vi "UMLEditor Main.vi"(1 "StartProject":string, 3 "StartTarget":string) -> ()   [LabVIEW 2020] (continued)
            n161 = call <resource>:"UndoEngine.vi"("Reference In"=w358, "Action"=enum16{"TakeSnapshot", "Undo", "Redo"}."TakeSnapshot", "Reset"=TRUE, "error in (no error)"=w357, "menu"=w356) -> ("Reference Out"=w355:refnum<class "Graph.lvclass">, "error out"=w354:errorcluster)  [unwired: 3 in, 10 out]
            n162 = Path To String(path=w368) -> (string=w367:string)
            n163 = call-dynamic "GetToolbarButtons.vi"("reference"=w355, "error in (no error)"=w354) -> ("AllToolbarButtons"=w351:T36[], "error out"=w353:errorcluster)  [unwired: 13 in, 3 out]
            n164 = case shown="False" w365 {
              tunnel: w367 -> [w373 _]
              tunnel: [w373 w374] -> w364
              tunnel: w363 -> [_ w374]
              frame False {
              }
              frame True {
              }
            }
            n165 = local write "GraphButtons"(T1."1" ("GraphButtons")) -> ()
            n166 = call <resource>:"UpdateToolbar.vi"("ToolbarButtons"=w351, "error in (no error)"=w353) -> ("error out"=w352:errorcluster)  [unwired: 17 in]
            n167 = property on="Diagram" class="Ring (strict)"("Tip Strip"=w364) -> ()  [unwired: 2 in, 2 out]
          }
          event "GraphButtons": Value Change {
            n168 = event-data() -> ()  [unwired: 7 out]
            n169 = call-dynamic "GetToolbarButtons.vi"("reference"=w378, "GraphButton"="GraphButtons", "error in (no error)"=w379) -> ("Type"=w376:T7, "error out"=w377:errorcluster)  [unwired: 12 in, 3 out]
            n170 = Bundle By Name(cluster=w381, "toolType"=w376) -> (w380:T5)
          }
          event "Help": Mouse Enter {
            n171 = event-data() -> ()  [unwired: 5 out]
            n172 = Unbundle By Name(w385) -> ("ToolHelp"=w384:bool)
            n173 = local read "Help"() -> (w383:bool)
            n174 = And(x=w384, y=w383) -> (x .and. y?=w382:bool)
            n175 = case shown="True" w382 {
              tunnel: w387 -> [w388 w391]
              tunnel: [w388 w390] -> w386
              frame False {
              }
              frame True {
                n176 = call <resource>:"ContextHelp_HelpTexts.vi"("HelpText (enum or string)"=ContextHelp_HelpTexts."Help" ("HelpText")) -> ("HelpOut"=w392:T38)  [unwired: 18 out]
                n177 = call <resource>:"ContextHelp_SendMessageToPopUp.vi"("PopUpMessage"=w392, "error in (no error)"=w391) -> ("error out"=w390:errorcluster)  [unwired: 1 in, 16 out]
              }
            }
          }
          event "Help": Value Change {
            n178 = event-data() -> ()  [unwired: 7 out]
            n179 = case shown="True" "Help" {
              tunnel: [ContextHelp_HelpTexts."None(Hide)" ("HelpText") ContextHelp_HelpTexts."Default" ("HelpText")] -> w395
              frame False {
              }
              frame True {
              }
            }
            n180 = call <resource>:"ContextHelp_HelpTexts.vi"("HelpText (enum or string)"=w395) -> ("HelpOut"=w398:T38)  [unwired: 18 out]
            n181 = call <resource>:"ContextHelp_SendMessageToPopUp.vi"("PopUpMessage"=w398, "error in (no error)"=w397) -> ("error out"=w396:errorcluster)  [unwired: 1 in, 16 out]
          }
          event "open": Value Change {
            n182 = event-data() -> ()  [unwired: 6 out]
            n183 = Bundle By Name(cluster=w402, "state"=UMLEditor_statesType."Open") -> (w403:T5)
          }
          event "Picture": Drag Enter {
            n184 = event-data() -> ("Coords"=w406:T39, "Available Data Names"=w405:string[])  [unwired: 8 out]
            n185 = stacked-sequence {
              tunnel: w406 -> [_]
              tunnel: w405 -> [_]
              frame #0 {
              }
            }
            n186 = event-data("Accepted?"=TRUE) -> ()  [unwired: 1 in, 1 out]
          }
          event "Picture": Mouse Down {
            # "Shift"
            n187 = event-data() -> ("Source"=w422:T40, "Button"=w416:u16, "Mods.Double Click"=w413:bool, "PlatMods.Ctrl"=w412:bool, "PlatMods.Shift"=w411:bool)  [unwired: 1 out]
            n188 = case shown="1, Default" w416 {
              selector: w416 -> [w453 _]
              tunnel: w422 -> [_ _]
              tunnel: w421 -> [w429 _]
              tunnel: [w462 w861] -> w420
              tunnel: w419 -> [w461 _]
              tunnel: w418 -> [w425 w860]
              tunnel: w410 -> [w452 w861]
              tunnel: [w454 w860] -> w417
              tunnel: w413 -> [w442 _]
              tunnel: w412 -> [w441 _]
              tunnel: w414 -> [_ _]
              tunnel: w411 -> [w433 _]
              frame 1, Default {
                n189 = local read "GraphButtons"() -> (w427:T1)
                n190 = call-dynamic "GetToolbarButtons.vi"("reference"=w429, "GraphButton"=w427, "error in (no error)"=w425) -> ("reference out"=w428:refnum<class "Graph.lvclass">, "Type"=w424:T7, "error out"=w426:errorcluster)  [unwired: 12 in, 2 out]
                n191 = property on="Picture" class="Pict"() -> ("Mouse"=w446:T41, "Draw Area Size"=w445:T42, "Origin"=w443:T43)  [unwired: 2 in, 2 out]
                n192 = Unbundle By Name(w452) -> ("graphics"=w436:refnum<class "Graphics.lvclass">, "SelectedNodes"=w448:refnum<class "AbstractNode.lvclass">[])
                n193 = Unbundle By Name(w452) -> ("HotSpotNode"=w430:refnum<class "AbstractNode.lvclass">, "HotSpotCursor"=w431:bool, "HotSpotFunction"=w432:T16, "zoom"=w455:dbl, "offset"=w457:T9)
                n194 = Unbundle By Name(w446) -> ("Mouse Position"=w458:cluster{"X":i32, "Y":i32})
                n195 = Array Size(array=w448) -> (size(s)=w450:i32)
                n196 = Greater?(x=w450, y=1) -> (0:w451:bool)
                n197 = Add(x=w457, y=w458) -> (x+y=w456:T9)
                n198 = call <resource>:"UMLEditor IsMouseOutsideDrawingArea.vi"("Mouse"=w446, "Draw Area Size"=w445, "Origin"=w443) -> ("OutsideDrawingArea"=w444:bool)  [unwired: 2 in, 14 out]
                n199 = Divide(x=w456, y=w455) -> (x/y=w440:T9)
                n200 = Bundle By Name(cluster=w452, "state"=UMLEditor_statesType."Repaint", "lastMousePoint"=w440) -> (w460:T5)
                n201 = call <resource>:"UMLEditor_FindObject.vi"("offset"=w440, "error in"=w426, "graphics"=w436, "graph"=w428) -> ("error out"=w439:errorcluster, "NodeFound"=w438:bool, "node"=w437:refnum<class "AbstractNode.lvclass">, "edge"=w435:refnum<class "AbstractEdge.lvclass">, "EdgeFound"=w434:bool)  [unwired: 2 in, 1 out]
                n202 = Tick Count (ms)() -> (millisecond timer value=w447:u32)
                n203 = case shown="False" w444 {
                  tunnel: w439 -> [w492 w859]
                  tunnel: w438 -> [w468 _]
                  tunnel: w434 -> [w477 _]
                  tunnel: w435 -> [w491 _]
                  tunnel: w437 -> [w490 _]
                  tunnel: [w489 w857] -> w462
                  tunnel: w461 -> [w487 _]
                  tunnel: w424 -> [w486 _]
                  tunnel: w428 -> [w485 _]
                  tunnel: w460 -> [w484 w858]
                  tunnel: w440 -> [w483 _]
                  tunnel: [w482 w859] -> w454
                  tunnel: w453 -> [w481 _]
                  tunnel: w451 -> [w480 _]
                  tunnel: w448 -> [w479 _]
                  tunnel: w447 -> [_ _]
                  tunnel: w445 -> [_ _]
                  tunnel: w442 -> [w469 _]
                  tunnel: w441 -> [w474 _]
                  tunnel: w436 -> [w472 _]
                  tunnel: w433 -> [w467 _]
                  tunnel: w432 -> [_ _]
                  tunnel: w431 -> [w465 _]
                  tunnel: w430 -> [w464 _]
                  tunnel: w427 -> [w463 _]
                  frame False {
                    n204 = Or(x=w468, y=w477) -> (x .or. y?=w476:bool)
                    n205 = And(x=w468, y=w467) -> (x .and. y?=w466:bool)
                    n206 = Compound Arithmetic op=AND(w469, w476) -> (w478:bool)
                    n207 = case shown="True" w478 {
                      tunnel: w492 -> [w509 w808]
                      tunnel: [w508 w807] -> w482
                      tunnel: w468 -> [w511 w806]
                      tunnel: w477 -> [w502 w801]
                      tunnel: w486 -> [w501 _]
                      tunnel: w484 -> [w514 w805]
                      tunnel: [w513 w804] -> w488
                      tunnel: w491 -> [w512 w803]
                      tunnel: w490 -> [w510 w802]
                      tunnel: w483 -> [w507 w799]
                      tunnel: w487 -> [w506 _]
                      tunnel: w485 -> [w505 _]
                      tunnel: w481 -> [_ _]
                      tunnel: w480 -> [w504 _]
                      tunnel: w479 -> [w503 _]
                      tunnel: UMLEditor_tooltype."None" ("t") -> [w500 _]
                      tunnel: w474 -> [w497 w800]
                      tunnel: [TRUE ("butDwn") w798] -> w473
                      tunnel: w472 -> [w498 _]
                      tunnel: w466 -> [w496 _]
                      tunnel: [w496 w798] -> w471
                      tunnel: [w497 w798] -> w470
                      tunnel: w469 -> [_ _]
                      tunnel: w465 -> [w495 _]
                      tunnel: w464 -> [w494 _]
                      tunnel: w463 -> [w493 _]
                      frame False {
                        # "Single Click"
                        n208 = case shown="True" w496 {
                          tunnel: w514 -> [w534 w786]
                          tunnel: [w533 w785] -> w513
                          tunnel: w512 -> [w532 _]
                          tunnel: w511 -> [w531 _]
                          tunnel: w510 -> [w530 w782]
                          tunnel: w509 -> [w529 w781]
                          tunnel: [w528 w781] -> w508
                          tunnel: w507 -> [w527 w784]
                          tunnel: w506 -> [w526 _]
                          tunnel: w505 -> [w525 _]
                          tunnel: w504 -> [w524 _]
                          tunnel: w503 -> [w523 w783]
                          tunnel: w502 -> [w522 _]
                          tunnel: w501 -> [w521 _]
                          tunnel: w500 -> [w519 _]
                          tunnel: w498 -> [w518 _]
                          tunnel: [_ w779] -> _
                          tunnel: w495 -> [w517 _]
                          tunnel: w494 -> [w516 _]
                          tunnel: w493 -> [w515 _]
                          frame False {
                            n209 = Select(t=w519, s=w522, f=w521) -> (s? t:f=w520:T7)
                            n210 = case shown="True" w517 {
                              tunnel: w534 -> [w551 w771]
                              tunnel: [w550 w770] -> w533
                              tunnel: w532 -> [w549 _]
                              tunnel: w531 -> [w548 _]
                              tunnel: w530 -> [w547 _]
                              tunnel: w529 -> [w546 w773]
                              tunnel: [w545 w772] -> w528
                              tunnel: w527 -> [w544 w769]
                              tunnel: w526 -> [w543 _]
                              tunnel: w525 -> [w542 _]
                              tunnel: w524 -> [w541 _]
                              tunnel: w523 -> [w540 _]
                              tunnel: w522 -> [w539 _]
                              tunnel: w520 -> [w538 _]
                              tunnel: w518 -> [w537 _]
                              tunnel: w517 -> [w536 _]
                              tunnel: w516 -> [_ w768]
                              tunnel: w515 -> [w535 _]
                              frame False {
                                n211 = case shown="\"None\", Default" w538 {
                                tunnel: w539 -> [w565 _ _]
                                tunnel: w551 -> [w564 w700 w747]
                                tunnel: [w563 w699 w746] -> w550
                                tunnel: w549 -> [w562 _ _]
                                tunnel: w548 -> [w561 w696 w744]
                                tunnel: w547 -> [w560 w695 w743]
                                tunnel: w546 -> [w559 w693 w742]
                                tunnel: [w558 w697 w741] -> w545
                                tunnel: w544 -> [w557 w694 w745]
                                tunnel: w543 -> [_ _ w740]
                                tunnel: w542 -> [w556 w692 w739]
                                tunnel: w541 -> [w555 _ _]
                                tunnel: w540 -> [w554 _ _]
                                tunnel: w537 -> [w553 _ _]
                                tunnel: w536 -> [w552 _ _]
                                tunnel: w535 -> [_ w691 w738]
                                frame "None", Default {
                                # "Select"
                                n212 = case shown="False" w565 {
                                tunnel: w564 -> [w574 w667]
                                tunnel: [w573 w666] -> w563
                                tunnel: w562 -> [_ w630]
                                tunnel: w561 -> [w575 _]
                                tunnel: w560 -> [w572 _]
                                tunnel: w559 -> [w571 w646]
                                tunnel: [w570 w646] -> w558
                                tunnel: w557 -> [w569 w641]
                                tunnel: w556 -> [_ _]
                                tunnel: w555 -> [w568 _]
                                tunnel: w554 -> [w567 _]
                                tunnel: w553 -> [_ w627]
                                tunnel: w552 -> [w566 _]
                                frame False {
                                n213 = case shown="True" w575 {
                                tunnel: w574 -> [w579 w625]
                                tunnel: [w584 w624] -> w573
                                tunnel: w572 -> [w585 _]
                                tunnel: w571 -> [w586 w621]
                                tunnel: [w583 w621] -> w570
                                tunnel: w569 -> [w582 w618]
                                tunnel: w568 -> [w581 _]
                                tunnel: w567 -> [w580 _]
                                tunnel: w566 -> [w576 _]
                                frame True {
                                # "Node Selected"
                                n214 = case shown="False" w576 {
                                frame False {
                                n215 = call <resource>:"UMLEditor_SetMouseCursor.vi"("CursorType"=UMLEditor_Cursortype."Move") -> ()  [unwired: 9 in, 2 out]
                                }
                                frame True {
                                }
                                }
                                n216 = Bundle By Name(cluster=w579, "state"=UMLEditor_statesType."Idle") -> (w577:T5)
                                n217 = case shown="False" w581 {
                                tunnel: w586 -> [w597 w601]
                                tunnel: w585 -> [w596 w600]
                                tunnel: w577 -> [w593 w599]
                                tunnel: [w592 w605] -> w584
                                tunnel: [w590 w601] -> w583
                                tunnel: w582 -> [w588 w604]
                                tunnel: w580 -> [_ w603]
                                frame False {
                                n218 = call-dynamic "getBounds.vi"("reference"=w596, "error in (no error)"=w597) -> ("reference out"=w595:refnum<class "AbstractNode.lvclass">, "bounds"=w594:T10, "error out"=w590:errorcluster)  [unwired: 15 in]
                                n219 = Build Array(w595) -> (w589:refnum<class "AbstractNode.lvclass">[])
                                n220 = Bundle By Name(cluster=w593, "selected"=UMLEditor_tooltype."Node" ("selcted"), "SelectedNodes"=w589, "dragStartBounds"=w594, "dragStartPoint"=w588, "newSelected"=TRUE, "lastMousePoint"=w588) -> (w592:T5)
                                }
                                frame True {
                                # "If many nodes allready selected move these"
                                n221 = Search 1D Array(1D array=w603, element=w600) -> (index of element=w602:i32)  [unwired: 1 out]
                                n222 = case shown="-1" w602 {
                                tunnel: w599 -> [w610 w617]
                                tunnel: [w609 w616] -> w605
                                tunnel: w604 -> [w608 w615]
                                tunnel: w600 -> [_ w612]
                                frame Default {
                                n223 = Bundle By Name(cluster=w610, "selected"=UMLEditor_tooltype."Node" ("selcted"), "dragStartPoint"=w608, "newSelected"=TRUE, "lastMousePoint"=w608) -> (w609:T5)
                                }
                                frame -1 {
                                n224 = Build Array(w612) -> (w611:refnum<class "AbstractNode.lvclass">[])
                                n225 = Bundle By Name(cluster=w617, "selected"=UMLEditor_tooltype."Node" ("selcted"), "dragStartPoint"=w615, "newSelected"=TRUE, "lastMousePoint"=w615, "SelectedNodes"=w611) -> (w616:T5)
                                }
                                }
                                }
                                }
                                }
                                frame False {
                                # "None Selected\nArea Select???"
                                n226 = Bundle By Name(cluster=w625, "selected"=UMLEditor_tooltype."None" ("selcted"), "SelectedNodes"=refnum<class "AbstractNode.lvclass">[] [], "dragStartBounds"=T10 {"x"=0.0, "y"=0.0, "width"=0.0, "height"=0.0}, "dragStartPoint"=w618, "rubberBandStart"=w618, "newSelected"=TRUE, "state"=UMLEditor_statesType."Idle", "lastMousePoint"=w618) -> (w624:T5)
                                }
                                }
                                }
                                frame True {
                                w663 = 25.0 ("y")
                                n227 = To More Specific Class(target class=refnum<class "GeneralPathEdge.lvclass"> refnum ("reference"), reference=w630) -> (specific class reference=w628:refnum<class "GeneralPathEdge.lvclass">)  [unwired: 1 in, 1 out]
                                n228 = call-dynamic "getPoints.vi"("reference"=w628, "error in (no error)"=w646) -> ("reference out"=w644:refnum<class "GeneralPathEdge.lvclass">, "points"=w642:T9[], "error out"=w645:errorcluster)  [unwired: 15 in]
                                n229 = Array Size(array=w642) -> (size(s)=w643:i32)
                                n230 = case shown="4" w643 {
                                tunnel: w642 -> [_ w676]
                                tunnel: w641 -> [_ w671]
                                tunnel: [_ w668] -> w636
                                frame Default {
                                }
                                frame 4 {
                                # "Egde selected"
                                n231 = Index Array(array=w676, index #1=1 ("index")) -> (element #1=w674:T9, element #2=w673:T9)  [unwired: 1 in]
                                n232 = Build Array(w674, w673) -> (w672:T9[])
                                n233 = call <resource>:"Point getDistanceToLine.vi"("point1"=w671, "line"=w672) -> ("minDistance"=w670:dbl)  [unwired: 1 in, 16 out]
                                n234 = Less?(x=w670, y=25.0) -> (x < y?=w668:bool)
                                }
                                }
                                n235 = Index Array(array=w642) -> (element=w662:T9)  [unwired: 1 in]
                                n236 = Delete From Array(array=w642) -> (deleted portion=w661:T9)  [unwired: 2 in, 1 out]
                                n237 = call-dynamic "GetTextPositions.vi"("reference"=w644, "GraphicsRef"=w627, "error in (no error)"=w645) -> ("reference out"=w654:refnum<class "GeneralPathEdge.lvclass">, "connectionPoints"=w653:T9[], "error out"=w655:errorcluster)  [unwired: 14 in]
                                n238 = Index Array(array=w653) -> (element=w652:T9)  [unwired: 1 in]
                                n239 = call <resource>:"Point getDistance.vi"("point1"=w662, "point2"=w641) -> ("distance"=w665:dbl)  [unwired: 1 in, 16 out]
                                n240 = call <resource>:"Point getDistance.vi"("point1"=w661, "point2"=w641) -> ("distance"=w664:dbl)  [unwired: 1 in, 16 out]
                                n241 = call-dynamic "getEnd.vi"("reference"=w654, "error in (no error)"=w655) -> ("reference out"=w659:refnum<class "GeneralPathEdge.lvclass">, "endNode"=w633:refnum<class "AbstractNode.lvclass">, "error out"=w660:errorcluster)  [unwired: 14 in, 1 out]
                                n242 = call <resource>:"Point getDistance.vi"("point1"=w652, "point2"=w641) -> ("distance"=w651:dbl)  [unwired: 1 in, 16 out]
                                n243 = Less?(x=w664, y=w663) -> (x < y?=w639:bool)
                                n244 = Less?(x=w665, y=w663) -> (x < y?=w638:bool)
                                n245 = Less?(x=w651, y=40.0) -> (x < y?=w640:bool)
                                n246 = call-dynamic "getStart.vi"("reference"=w659, "error in (no error)"=w660) -> ("startNode"=w632:refnum<class "AbstractNode.lvclass">, "error out"=w658:errorcluster)  [unwired: 14 in, 2 out]
                                n247 = Select(t=w633, s=w639, f=w632) -> (s? t:f=w649:refnum<class "AbstractNode.lvclass">)
                                n248 = Unbundle By Name(w658) -> ("status"=w657:bool)
                                n249 = Build Array(w633, w632) -> (w631:refnum<class "AbstractNode.lvclass">[])
                                n250 = Compound Arithmetic op=OR(w636, w638, w639, w640) -> (w637:bool)
                                n251 = Build Array(w649) -> (w635:refnum<class "AbstractNode.lvclass">[])
                                n252 = Compound Arithmetic op=AND(w637, invert w657) -> (w656:bool)
                                n253 = Select(t=w631, s=w636, f=w635) -> (s? t:f=w634:refnum<class "AbstractNode.lvclass">[])
                                n254 = Select(t=refnum<class "AbstractNode.lvclass">[] [], s=w640, f=w634) -> (s? t:f=w647:refnum<class "AbstractNode.lvclass">[])
                                n255 = case shown="True" w656 {
                                tunnel: w667 -> [w683 w688]
                                tunnel: [w682 w687] -> w666
                                tunnel: w630 -> [w679 w684]
                                tunnel: w641 -> [w678 _]
                                tunnel: w647 -> [w677 _]
                                frame True {
                                n256 = Bundle By Name(cluster=w683, "selected"=UMLEditor_tooltype."Edge" ("selcted"), "selectedEdge"=w679, "dragStartPoint"=w678, "newSelected"=TRUE, "SelectedNodes"=w677) -> (w682:T5)
                                }
                                frame False {
                                n257 = Bundle By Name(cluster=w688, "selected"=UMLEditor_tooltype."Edge" ("selcted"), "selectedEdge"=w684, "newSelected"=TRUE) -> (w687:T5)
                                }
                                }
                                }
                                }
                                }
                                frame "Node" {
                                # "Node Tool"
                                n258 = call-dynamic "CreateToolbarObject.vi"("reference in"=w692, "GraphButton"=w691, "error in (no error)"=w693) -> ("Node"=w689:refnum<class "AbstractNode.lvclass">, "error out"=w690:errorcluster)  [unwired: 11 in, 4 out]
                                n259 = call-dynamic "add.vi"("reference"=w692, "node"=w689, "point"=w694, "error in (no error)"=w690) -> ("added"=w701:bool, "error out"=w698:errorcluster)  [unwired: 13 in, 1 out]
                                n260 = case shown="False" w701 {
                                tunnel: w700 -> [w709 w729]
                                tunnel: [w708 w727] -> w699
                                tunnel: w698 -> [w704 w737]
                                tunnel: w689 -> [w702 w736]
                                tunnel: w694 -> [w706 w725]
                                tunnel: [w705 w730] -> w697
                                tunnel: w696 -> [w710 _]
                                tunnel: w695 -> [w707 _]
                                frame False {
                                n261 = call-dynamic "Destroy.vi"("reference"=w702, "error in (no error)"=w704) -> ("error out"=w703:errorcluster)  [unwired: 16 in, 1 out]
                                n262 = case shown="True" w710 {
                                tunnel: w709 -> [w712 w721]
                                tunnel: [w712 w720] -> w708
                                tunnel: w703 -> [w711 w723]
                                tunnel: w707 -> [_ w715]
                                tunnel: w706 -> [_ w717]
                                tunnel: [w711 w719] -> w705
                                frame False {
                                }
                                frame True {
                                # "Node Found"
                                n263 = call-dynamic "getBounds.vi"("reference"=w715, "error in (no error)"=w723) -> ("bounds"=w722:T10, "error out"=w719:errorcluster)  [unwired: 15 in, 1 out]
                                n264 = Build Array(w715) -> (w718:refnum<class "AbstractNode.lvclass">[])
                                n265 = local write "GraphButtons"(T1."1" ("GraphButtons")) -> ()
                                n266 = Bundle By Name(cluster=w721, "selected"=UMLEditor_tooltype."Node" ("selcted"), "SelectedNodes"=w718, "dragStartBounds"=w722, "dragStartPoint"=w717, "lastMousePoint"=w717, "newSelected"=TRUE, "toolType"=UMLEditor_tooltype."None") -> (w720:T5)
                                }
                                }
                                }
                                frame True {
                                # "Added"
                                n267 = call-dynamic "getBounds.vi"("reference"=w736, "error in (no error)"=w737) -> ("reference out"=w734:refnum<class "AbstractNode.lvclass">, "bounds"=w735:T10, "error out"=w731:errorcluster)  [unwired: 15 in]
                                n268 = Build Array(w734) -> (w726:refnum<class "AbstractNode.lvclass">[])
                                n269 = Bundle By Name(cluster=w729, "selected"=UMLEditor_tooltype."Node" ("selcted"), "SelectedNodes"=w726, "dragStartBounds"=w735, "dragStartPoint"=w725, "lastMousePoint"=w725) -> (w728:T5)
                                n270 = call <resource>:"UMLEditor setDiagramInfo.vi"("error in (no error)"=w731, "localVariablesIn"=w728, "action"=enum16{"Name/Dir", "Unsaved", "Saved"}."Unsaved") -> ("localVariablesOut"=w727:T5, "error out"=w730:errorcluster)  [unwired: 2 in, 13 out]
                                }
                                }
                                }
                                frame "Edge" {
                                # "Edge Tool"
                                n271 = case shown="True" w744 {
                                tunnel: w747 -> [w750 w761]
                                tunnel: [w749 w760] -> w746
                                tunnel: w745 -> [_ w759]
                                tunnel: w743 -> [_ w758]
                                tunnel: w742 -> [w752 w757]
                                tunnel: [w752 w755] -> w741
                                tunnel: w740 -> [_ _]
                                tunnel: w739 -> [_ w754]
                                tunnel: w738 -> [_ w753]
                                frame False {
                                n272 = local write "GraphButtons"(T1."1" ("GraphButtons")) -> ()
                                n273 = Bundle By Name(cluster=w750, "toolType"=UMLEditor_tooltype."None") -> (w749:T5)
                                }
                                frame True {
                                n274 = call-dynamic "AllowEdgeStartCheck.vi"("reference in"=w754, "EdgeStartNode"=w758, "GraphButton"=w753, "error in (no error)"=w757) -> ("Allowed"=w756:bool, "error out"=w755:errorcluster)  [unwired: 13 in, 1 out]
                                n275 = case shown="True" w756 {
                                tunnel: w761 -> [w762 w767]
                                tunnel: [w762 w766] -> w760
                                tunnel: w759 -> [_ w765]
                                frame False {
                                }
                                frame True {
                                n276 = Bundle By Name(cluster=w767, "rubberBandStart"=w765, "selected"=UMLEditor_tooltype."Edge" ("selcted"), "state"=UMLEditor_statesType."Idle") -> (w766:T5)
                                }
                                }
                                }
                                }
                                }
                                }
                              }
                              frame True {
                                n277 = call-dynamic "getBounds.vi"("reference"=w768, "error in (no error)"=w773) -> ("reference out"=w777:refnum<class "AbstractNode.lvclass">, "bounds"=w776:T10, "error out"=w772:errorcluster)  [unwired: 15 in]
                                n278 = Build Array(w777) -> (w774:refnum<class "AbstractNode.lvclass">[])
                                n279 = Bundle By Name(cluster=w771, "selected"=UMLEditor_tooltype."Node" ("selcted"), "SelectedNodes"=w774, "dragStartBounds"=w776, "dragStartPoint"=w769, "newSelected"=TRUE, "lastMousePoint"=w769) -> (w770:T5)
                              }
                            }
                          }
                          frame True {
                            # "Shift Click"
                            n280 = Search 1D Array(1D array=w783, element=w782) -> (index of element=w791:i32)  [unwired: 1 in]
                            n281 = case shown="0, Default" w791 {
                              selector: w791 -> [w792 _]
                              tunnel: w783 -> [w794 w797]
                              tunnel: w782 -> [_ w796]
                              tunnel: [w793 w795] -> w780
                              frame 0, Default {
                                n282 = Delete From Array(array=w794, index=w792) -> (array with subset deleted=w793:refnum<class "AbstractNode.lvclass">[])  [unwired: 1 in, 1 out]
                              }
                              frame -1 {
                                n283 = Build Array (concatenate)(w797, w796) -> (w795:refnum<class "AbstractNode.lvclass">[])
                              }
                            }
                            n284 = Array Size(array=w780) -> (size(s)=w779:i32)
                            n285 = Bundle By Name(cluster=w786, "selected"=UMLEditor_tooltype."Node" ("selcted"), "SelectedNodes"=w780, "dragStartBounds"=T10 {"x"=nan, "y"=nan, "width"=nan, "height"=nan}, "dragStartPoint"=T9 {"x"=nan, "y"=nan}, "newSelected"=TRUE, "lastMousePoint"=w784) -> (w785:T5)
                          }
                        }
                      }
                      frame True {
                        w798 = FALSE ("butDwn")
                        # "DblClick"
                        n286 = case shown="True" w801 {
                          tunnel: w808 -> [w817 w851]
                          tunnel: [w816 w851] -> w807
                          tunnel: w806 -> [w815 _]
                          tunnel: w805 -> [w814 w853]
                          tunnel: [w813 w852] -> w804
                          tunnel: w803 -> [w812 w850]
                          tunnel: w802 -> [w811 _]
                          tunnel: w800 -> [w810 _]
                          tunnel: w799 -> [w809 _]
                          frame False {
                            n287 = case shown="False" w815 {
                              tunnel: w817 -> [w818 w823]
                              tunnel: [w818 w822] -> w816
                              tunnel: w814 -> [w819 w826]
                              tunnel: [w819 w825] -> w813
                              tunnel: w812 -> [_ _]
                              tunnel: w811 -> [_ w820]
                              tunnel: w810 -> [_ w824]
                              tunnel: w809 -> [_ w821]
                              frame False {
                              }
                              frame True {
                                # "Node Found"
                                n288 = case shown="True" w824 {
                                tunnel: w826 -> [w831 w838]
                                tunnel: [w830 w837] -> w825
                                tunnel: w820 -> [w828 _]
                                tunnel: w823 -> [w827 w842]
                                tunnel: [w827 w841] -> w822
                                tunnel: w821 -> [_ w840]
                                tunnel: w820 -> [_ w839]
                                frame False {
                                n289 = Build Array(w828) -> (w829:refnum<class "AbstractNode.lvclass">[])
                                n290 = Bundle By Name(cluster=w831, "selected"=UMLEditor_tooltype."Node" ("selcted"), "SelectedNodes"=w829, "state"=UMLEditor_statesType."EditSelected") -> (w830:T5)
                                }
                                frame True {
                                n291 = call-dynamic "GetContextHelpInfo.vi"("reference"=w839, "MousePos"=w840, "error in (no error)"=w842) -> ("ContextHelpInfo"=w836:variant, "error out"=w841:errorcluster)  [unwired: 13 in, 2 out]
                                n292 = Variant To Data(type=path "", Variant=w836) -> (error out=w834:errorcluster)  [unwired: 1 in, 1 out]
                                n293 = case shown="No Error" w834 {
                                tunnel: w838 -> [w847 w849]
                                tunnel: [w846 w849] -> w837
                                tunnel: w836 -> [w843 _]
                                frame No Error {
                                # "Ctrl-Key down\nSo lets open the method"
                                n294 = Bundle By Name(cluster=T12 {"Command"=enum."OpenFile", "CommandData"=variant} ("FlattenCommandSettings"), "CommandData"=w843) -> (w844:T12)
                                n295 = Bundle By Name(cluster=w847, "state"=UMLEditor_statesType."ExecuteCommand", "FlattenCommandSettings"=w844) -> (w846:T5)
                                }
                                frame Error {
                                }
                                }
                                }
                                }
                              }
                            }
                          }
                          frame True {
                            # "Edge Found"
                            n296 = Bundle By Name(cluster=w853, "selected"=UMLEditor_tooltype."Edge" ("selcted"), "selectedEdge"=w850, "state"=UMLEditor_statesType."EditSelected") -> (w852:T5)
                          }
                        }
                      }
                    }
                    n297 = Bundle By Name(cluster=w488, "butDwn"=w473, "ShiftDown"=w471, "CtrlDown"=w470) -> (w489:T5)
                  }
                  frame True {
                    # "SCROLLING"
                    n298 = Bundle By Name(cluster=w858, "state"=UMLEditor_statesType."Idle") -> (w857:T5)
                  }
                }
              }
              frame 0, 2 {
              }
            }
            n299 = property on="ClassAggregationDialog" class="Clust (strict)"() -> ("Visible"=w415:bool)  [unwired: 2 in, 2 out]
            n300 = case shown="True" w415 {
              frame False {
              }
              frame True {
                n301 = property on="ClassAggregationDialog" class="Clust (strict)"("Visible"=FALSE) -> ()  [unwired: 2 in, 2 out]
              }
            }
          }
          event "Picture": Mouse Enter {
            n302 = event-data() -> ()  [unwired: 5 out]
            n303 = call <resource>:"UMLEditor_SetMouseCursor.vi"("CursorType"=UMLEditor_Cursortype."Arrow") -> ("error out"=w863:errorcluster)  [unwired: 9 in, 1 out]
            n304 = property on="Picture" class="Pict"(error in=w863, "Cursor"=0) -> ()  [unwired: 1 in, 2 out]
          }
          event "Picture": Mouse Leave {
            n305 = event-data() -> ()  [unwired: 5 out]
            n306 = Unbundle By Name(w872) -> ("butDwn"=w871:bool)
            n307 = call <resource>:"UMLEditor_SetMouseCursor.vi"("CursorType"=UMLEditor_Cursortype."Arrow") -> ()  [unwired: 9 in, 2 out]
            n308 = Select(t=UMLEditor_statesType."Repaint" ("state"), s=w871, f=UMLEditor_statesType."Idle" ("state")) -> (s? t:f=w870:T6)
            n309 = Bundle By Name(cluster=w872, "state"=w870) -> (w873:T5)
          }
          event "Picture": Mouse Up {
            w905 = T9 {"x"=nan, "y"=nan} ("rubberBandStart")
            w880 = FALSE ("b_dwn")
            n310 = event-data() -> ("Mods.Double Click"=w893:bool, "Coords"=w888:T39)  [unwired: 1 out]
            n311 = Unbundle By Name(w875) -> ("lastMousePoint"=w879:T9, "rubberBandStart"=w901:T9, "selected"=w896:T7, "offset"=w884:T9, "zoom"=w882:dbl)
            n312 = Unbundle By Name(w875) -> ("SelectedNodes"=w894:refnum<class "AbstractNode.lvclass">[])
            n313 = Unbundle By Name(w875) -> ("HotSpotCursor"=w887:bool, "HotSpotFunction"=w886:T16)
            n314 = Unbundle By Name(w875) -> ("CONNECT_THRESHOLD"=w900:i32)
            n315 = property on="Picture" class="Pict"() -> ("Mouse"=w878:T41, "Draw Area Size"=w890:T42, "Origin"=w889:T43)  [unwired: 2 in, 2 out]
            n316 = Unbundle By Name(w878) -> ("Mouse Position"=w885:cluster{"X":i32, "Y":i32})
            n317 = call <resource>:"UMLEditor_SetMouseCursor.vi"("CursorType"=UMLEditor_Cursortype."Arrow") -> ()  [unwired: 9 in, 2 out]
            n318 = Tick Count (ms)() -> (millisecond timer value=w892:u32)
            n319 = Add(x=w885, y=w884) -> (x+y=w883:T9)
            n320 = call <resource>:"UMLEditor IsMouseOutsideDrawingArea.vi"("Mouse"=w878, "Draw Area Size"=w890, "Origin"=w889) -> ("OutsideDrawingArea"=w891:bool)  [unwired: 2 in, 14 out]
            n321 = call <resource>:"Point getValues.vi"("point2D"=w901) -> ("valid"=w903:bool)  [unwired: 18 out]
            n322 = Divide(x=w883, y=w882) -> (x/y=w881:T9)
            n323 = case shown="False" w891 {
              tunnel: w903 -> [w923 _]
              tunnel: w902 -> [w922 w1197]
              tunnel: w901 -> [w921 _]
              tunnel: w900 -> [w920 _]
              tunnel: [w909 w1196] -> w899
              tunnel: w898 -> [w919 _]
              tunnel: [w918 w1197] -> w897
              tunnel: w896 -> [w917 _]
              tunnel: w875 -> [w916 w1196]
              tunnel: UMLEditor_tooltype."None" ("y") -> [w915 _]
              tunnel: w894 -> [w914 _]
              tunnel: w893 -> [w913 _]
              tunnel: w892 -> [w912 _]
              tunnel: w888 -> [w911 _]
              tunnel: w887 -> [w910 _]
              tunnel: w886 -> [w908 _]
              tunnel: w881 -> [w907 _]
              tunnel: w879 -> [w906 _]
              frame False {
                n324 = case shown="False" w910 {
                  tunnel: w923 -> [w939 _]
                  tunnel: w922 -> [w938 w1151]
                  tunnel: w921 -> [w937 _]
                  tunnel: w920 -> [w936 _]
                  tunnel: w919 -> [w934 w1147]
                  tunnel: [w933 w1154] -> w918
                  tunnel: w917 -> [w932 _]
                  tunnel: w916 -> [w931 w1153]
                  tunnel: w915 -> [w930 _]
                  tunnel: w914 -> [w929 w1150]
                  tunnel: w913 -> [w928 _]
                  tunnel: w912 -> [w927 _]
                  tunnel: w911 -> [w926 _]
                  tunnel: [w935 w1152] -> w909
                  tunnel: w908 -> [_ w1149]
                  tunnel: w907 -> [w925 w1148]
                  tunnel: w906 -> [w924 _]
                  frame False {
                    n325 = case shown="False" w939 {
                      tunnel: w938 -> [w952 w1047]
                      tunnel: w931 -> [w953 w1046]
                      tunnel: w937 -> [_ w1042]
                      tunnel: w936 -> [_ w1045]
                      tunnel: w931 -> [w949 w1040]
                      tunnel: [w948 w1044] -> w935
                      tunnel: w934 -> [w950 w1043]
                      tunnel: [w951 w1041] -> w933
                      tunnel: w932 -> [w947 w1039]
                      tunnel: w930 -> [w944 _]
                      tunnel: w929 -> [w943 _]
                      tunnel: w928 -> [w942 _]
                      tunnel: w927 -> [_ _]
                      tunnel: w926 -> [_ w1038]
                      tunnel: w925 -> [w941 w1037]
                      tunnel: w924 -> [w940 _]
                      frame False {
                        # "Try to lock Assoc to grid is offset is used"
                        n326 = Not Equal?(x=w947, y=w944) -> (x != y?=w946:bool)
                        n327 = And(x=w946, y=w942) -> (x .and. y?=w945:bool)
                        n328 = case shown="False" w945 {
                          tunnel: w947 -> [w964 w1026]
                          tunnel: w953 -> [w963 _]
                          tunnel: w952 -> [w962 w1028]
                          tunnel: [w961 w1028] -> w951
                          tunnel: w950 -> [w960 _]
                          tunnel: w949 -> [w959 w1030]
                          tunnel: [w958 w1029] -> w948
                          tunnel: w943 -> [w957 w1027]
                          tunnel: w941 -> [w956 _]
                          tunnel: w941 -> [w955 _]
                          tunnel: w940 -> [w954 _]
                          frame False {
                            n329 = case shown="\"Edge\"" w964 {
                              tunnel: w963 -> [_ w977 _]
                              tunnel: w962 -> [w966 w976 w984]
                              tunnel: [w966 w974 w985] -> w961
                              tunnel: w960 -> [_ w973 w982]
                              tunnel: w959 -> [w965 w969 w987]
                              tunnel: [w965 w968 w986] -> w958
                              tunnel: w957 -> [_ _ w981]
                              tunnel: w956 -> [_ _ w983]
                              tunnel: w955 -> [_ _ w980]
                              tunnel: w954 -> [_ _ w979]
                              frame Default {
                              }
                              frame "Edge" {
                                n330 = Unbundle By Name(w977) -> ("selectedEdge"=w975:refnum<class "AbstractEdge.lvclass">, "graphics"=w972:refnum<class "Graphics.lvclass">, "grid"=w971:refnum<class "Grid.lvclass">)
                                n331 = call-dynamic "Layout.vi"("reference"=w975, "graph"=w973, "graphics"=w972, "grid"=w971, "error in (no error)"=w976) -> ("error out"=w974:errorcluster)  [unwired: 13 in, 1 out]
                                n332 = Bundle By Name(cluster=w969, "SelectedNodes"=refnum<class "AbstractNode.lvclass">[] [], "state"=UMLEditor_statesType."Repaint") -> (w968:T5)
                              }
                              frame "Node" {
                                n333 = case shown="True" TRUE {
                                tunnel: [w989 w1000] -> w985
                                tunnel: w984 -> [w989 w999]
                                tunnel: w983 -> [_ w998]
                                tunnel: w982 -> [_ w996]
                                tunnel: w981 -> [_ w990]
                                frame False {
                                }
                                frame True {
                                n334 = for {
                                tunnel: w998 -> [w1011]
                                tunnel: w996 -> [w1009]
                                shift-right: [w1010] -> w997
                                shift-left: w999 -> [w1012]
                                tunnel: w990 -> [w1008] mode=indexing
                                shift-right: [w1006] -> w994
                                shift-left: FALSE -> [w1007]
                                shift-right: [w1002] -> w992
                                shift-left: refnum<class "AbstractNode.lvclass"> refnum ("container") -> [w1003]
                                tunnel: w990 -> [w1001]
                                n335 = call-dynamic "contains.vi"("reference"=w1009, "node"=w1008, "point2D"=w1011, "error in (no error)"=w1012, "IgnoreNodes"=w1001) -> ("contains"=w1005:bool, "container"=w1004:refnum<class "AbstractNode.lvclass">, "error out"=w1010:errorcluster)  [unwired: 11 in, 1 out]
                                n336 = Or(x=w1007, y=w1005) -> (x .or. y?=w1006:bool)
                                n337 = Select(t=w1004, s=w1005, f=w1003) -> (s? t:f=w1002:refnum<class "AbstractNode.lvclass">)
                                }
                                n338 = case shown="True" w994 {
                                tunnel: [w1013 w1014] -> w995
                                tunnel: w990 -> [_ w1019]
                                tunnel: w997 -> [w1013 w1018]
                                tunnel: w992 -> [_ w1017]
                                tunnel: w996 -> [_ w1015]
                                frame False {
                                }
                                frame True {
                                n339 = for {
                                tunnel: w1019 -> [w1024] mode=indexing
                                shift-right: [w1023] -> w1016
                                shift-left: w1018 -> [w1022]
                                tunnel: [w1021] -> _
                                tunnel: w1017 -> [w1020]
                                n340 = call-dynamic "addNode.vi"("reference"=w1020, "node"=w1024, "error in (no error)"=w1022) -> ("added"=w1021:bool, "error out"=w1023:errorcluster)  [unwired: 14 in, 1 out]
                                }
                                n341 = call-dynamic "RearrangeNodes.vi"("reference in"=w1015, "error in (no error)"=w1016) -> ("error out"=w1014:errorcluster)  [unwired: 16 in, 1 out]
                                }
                                }
                                n342 = call-dynamic "layout.vi"("reference"=w996, "LayoutNodes(Empty=All)"=w990, "error in (no error)"=w995) -> ("error out"=w1000:errorcluster)  [unwired: 15 in, 1 out]
                                }
                                }
                                n343 = Not Equal?(x=w979, y=w980) -> ()  [unwired: 1 out]
                                n344 = Bundle By Name(cluster=w987, "state"=UMLEditor_statesType."Repaint") -> (w986:T5)
                              }
                            }
                          }
                          frame True {
                            n345 = case shown="True" FALSE {
                              tunnel: w1030 -> [w1031 w1035]
                              tunnel: [w1031 w1034] -> w1029
                              tunnel: w1027 -> [_ w1033]
                              tunnel: w1026 -> [_ w1032]
                              frame False {
                              }
                              frame True {
                                (unwired) UMLEditor_tooltype."Node" ("selcted")
                                n346 = Bundle By Name(cluster=w1035, "selected"=w1032, "SelectedNodes"=w1033, "state"=UMLEditor_statesType."EditSelected") -> (w1034:T5)
                              }
                            }
                          }
                        }
                      }
                      frame True {
                        n347 = case shown="Default" w1039 {
                          tunnel: w1047 -> [w1072 w1093]
                          tunnel: w1046 -> [_ w1092]
                          tunnel: w1045 -> [_ w1089]
                          tunnel: [w1069 w1088] -> w1044
                          tunnel: w1043 -> [w1071 w1074]
                          tunnel: w1042 -> [w1050 w1086]
                          tunnel: [w1063 w1083] -> w1041
                          tunnel: w1040 -> [w1070 w1080]
                          tunnel: w1038 -> [_ w1076]
                          tunnel: w1037 -> [w1048 w1075]
                          frame "None", "Node" {
                            n348 = Unbundle(w1050) -> ("x"=w1058:dbl, "y"=w1054:dbl)
                            n349 = Unbundle(w1048) -> ("x"=w1057:dbl, "y"=w1053:dbl)
                            n350 = Max & Min(x=w1058, y=w1057) -> (max(x,y)=w1056:dbl, min(x,y)=w1055:dbl)
                            n351 = Max & Min(x=w1054, y=w1053) -> (max(x,y)=w1052:dbl, min(x,y)=w1051:dbl)
                            n352 = Subtract(x=w1056, y=w1055) -> (x-y=w1060:dbl)
                            n353 = Subtract(x=w1052, y=w1051) -> (x-y=w1059:dbl)
                            n354 = Bundle By Name(cluster=T10 {"x"=0.0, "y"=0.0, "width"=0.0, "height"=0.0} ("rectangle"), "x"=w1055, "y"=w1051, "width"=w1060, "height"=w1059) -> (w1049:T10)
                            n355 = call-dynamic "findNodes.vi"("reference"=w1071, "bounds"=w1049, "error in (no error)"=w1072) -> ("Nodes"=w1064:refnum<class "AbstractNode.lvclass">[], "AnyFound"=w1068:bool, "error out"=w1063:errorcluster)  [unwired: 12 in, 2 out]
                            n356 = Select(t=UMLEditor_tooltype."Node" ("selcted"), s=w1068, f=UMLEditor_tooltype."None" ("selcted")) -> (s? t:f=w1067:T7)
                            n357 = Bundle By Name(cluster=w1070, "SelectedNodes"=w1064, "selected"=w1067, "state"=UMLEditor_statesType."Repaint") -> (w1069:T5)
                          }
                          frame Default {
                            n358 = local read "GraphButtons"() -> (w1073:T1)
                            n359 = disable-structure shown="Enabled" {
                              disable-tunnel: w1093 -> [w1100 w1106]
                              disable-tunnel: w1092 -> [w1099 _]
                              disable-tunnel: [w1096 w1102] -> w1091
                              disable-tunnel: [w1095 w1103] -> w1084
                              disable-tunnel: [w1094 w1101] -> w1077
                              disable-tunnel: w1074 -> [_ w1105]
                              disable-tunnel: w1073 -> [_ w1104]
                              frame Disabled {
                                n360 = call <resource>:"UMLEditor ToolBarSettings.vi"("localVariables"=w1099, "error in (no error)"=w1100) -> ("tools"=w1094:T44, "prototypeEdge"=w1098:refnum<class "AbstractEdge.lvclass">, "error out"=w1097:errorcluster)  [unwired: 2 in, 13 out]
                                n361 = call-dynamic "clone.vi"("reference"=w1098, "error in (no error)"=w1097) -> ("clonedEdge"=w1095:refnum<class "AbstractEdge.lvclass">, "error out"=w1096:errorcluster)  [unwired: 15 in, 1 out]
                              }
                              frame Enabled {
                                n362 = call-dynamic "CreateToolbarObject.vi"("reference in"=w1105, "GraphButton"=w1104, "error in (no error)"=w1106) -> ("Edge"=w1103:refnum<class "AbstractEdge.lvclass">, "ButtonNameCompressed)"=w1101:string, "error out"=w1102:errorcluster)  [unwired: 11 in, 3 out]
                              }
                            }
                            n363 = call <resource>:"Point getDistance.vi"("point1"=w1086, "point2"=w1075, "error in (no error)"=w1091) -> ("distance"=w1090:dbl, "error out"=w1087:errorcluster)  [unwired: 15 out]
                            n364 = Greater?(x=w1090, y=w1089) -> (0:w1081:bool)
                            n365 = case shown="True" w1081 {
                              tunnel: w1087 -> [w1107 w1115]
                              tunnel: w1074 -> [_ w1114]
                              tunnel: w1086 -> [_ w1113]
                              tunnel: w1075 -> [_ w1112]
                              tunnel: [w1107 w1111] -> w1085
                              tunnel: w1084 -> [_ w1110]
                              tunnel: [FALSE ("connected") w1109] -> w1082
                              frame False {
                              }
                              frame True {
                                n366 = call-dynamic "connect.vi"("reference"=w1114, "egde"=w1110, "p1"=w1113, "p2"=w1112, "error in (no error)"=w1115) -> ("connected"=w1109:bool, "error out"=w1111:errorcluster)  [unwired: 12 in, 1 out]
                              }
                            }
                            n367 = Bundle By Name(cluster=w1080, "state"=UMLEditor_statesType."Repaint") -> (w1078:T5)
                            n368 = case shown="True" w1082 {
                              tunnel: [w1117 w1130] -> w1088
                              tunnel: w1085 -> [w1121 w1125]
                              tunnel: w1084 -> [w1120 w1127]
                              tunnel: [w1119 w1129] -> w1083
                              tunnel: w1078 -> [w1118 w1128]
                              tunnel: w1074 -> [_ w1126]
                              tunnel: w1077 -> [_ w1123]
                              tunnel: w1076 -> [_ w1122]
                              frame False {
                                n369 = call-dynamic "Destroy.vi"("reference"=w1120, "error in (no error)"=w1121) -> ("error out"=w1119:errorcluster)  [unwired: 17 in]
                                n370 = Bundle By Name(cluster=w1118, "selected"=UMLEditor_tooltype."None" ("selcted")) -> (w1117:T5)
                              }
                              frame True {
                                n371 = case shown="Default" w1123 {
                                tunnel: w1127 -> [w1138 w1146]
                                tunnel: w1126 -> [w1139 w1145]
                                tunnel: w1125 -> [w1140 w1144]
                                tunnel: [w1137 w1143] -> w1124
                                tunnel: w1122 -> [w1135 _]
                                frame "Aggregation", "CompositeAggregation" {
                                n372 = call <resource>:"UMLEditor ShowAggregationDialog.vi"("graph"=w1139, "ClassAggregation"=w1138, "error in (no error)"=w1140) -> ("Show"=w1136:bool, "error out"=w1137:errorcluster)  [unwired: 15 out]
                                n373 = case shown="True" w1136 {
                                tunnel: w1135 -> [_ w1142]
                                frame False {
                                }
                                frame True {
                                n374 = call <resource>:"UMLEditor_AggregationClusterDialogControl.vi"("Position"=w1142, "Action(SelectSelect)"=T19."CreateAggregation") -> ()  [unwired: 7 in, 11 out]
                                }
                                }
                                }
                                frame Default {
                                n375 = call <resource>:"UMLEditor CreateNoteText.vi"("graph"=w1145, "NoteEdge?"=w1146, "error in (no error)"=w1144) -> ("error out"=w1143:errorcluster)  [unwired: 16 out]
                                }
                                }
                                n376 = Bundle By Name(cluster=w1128, "modified"=TRUE, "selected"=UMLEditor_tooltype."Edge" ("selcted"), "selectedEdge"=w1127) -> (w1131:T5)
                                n377 = call <resource>:"UMLEditor setDiagramInfo.vi"("error in (no error)"=w1124, "localVariablesIn"=w1131, "action"=enum16{"Name/Dir", "Unsaved", "Saved"}."Unsaved") -> ("localVariablesOut"=w1130:T5, "error out"=w1129:errorcluster)  [unwired: 2 in, 13 out]
                              }
                            }
                          }
                        }
                      }
                    }
                  }
                  frame True {
                    n378 = Bundle By Name(cluster=w1153, "HotSpotCursor"=FALSE) -> (w1155:T5)
                    n379 = case shown="\"Expand\", \"Collaps\"" w1149 {
                      tunnel: w1155 -> [w1159 w1174]
                      tunnel: [w1163 w1173] -> w1154
                      tunnel: [w1158 w1172] -> w1152
                      tunnel: w1151 -> [w1165 w1171]
                      tunnel: w1149 -> [_ w1170]
                      tunnel: w1150 -> [w1162 w1169]
                      tunnel: w1148 -> [w1157 w1167]
                      tunnel: w1147 -> [w1164 w1166]
                      frame Default {
                        n380 = call-dynamic "layout.vi"("reference"=w1164, "LayoutNodes(Empty=All)"=w1162, "error in (no error)"=w1165) -> ("error out"=w1163:errorcluster)  [unwired: 15 in, 1 out]
                        n381 = Bundle By Name(cluster=w1159, "newSelected"=FALSE ("HotSpotCursor"), "state"=UMLEditor_statesType."Repaint", "lastMousePoint"=w1157) -> (w1158:T5)
                      }
                      frame "Expand", "Collaps" {
                        n382 = Array Size(array=w1169) -> (size(s)=w1168:i32)
